vi "Tester - Index First and Last Elements.vi"() -> ()   [LabVIEW 2026, in "RSysUtils Array.lvlib"]
uses:
  RSysUtils Array.lvlib
  fdb9e6c0-975f-44e2-ba30-bd03142f5d50.vi
  b5e11ca3-2994-41fd-9918-31737f74fe56.vi
  f58beb1a-473f-4e9f-bfc2-1733d708c953.vi
  5ddec0b6-ee56-4581-aaaf-1957dd87ccd5.vi
  00215f05-ef31-4d06-8534-21c6b446a682.vi
  7647355d-b8e7-4a93-9c24-6d2a4ea71276.vi
  75d32098-2e7f-4ed5-a06b-df6319fe105d.vi
  2febbabd-baec-49ef-bef3-c8b34b704352.vi
  cc8c92ee-e4ab-4953-afd2-d877638164e4.vi
  083ab0fe-1952-43f6-ad3a-e45cd4cdc5d8.vi
  f95bf693-d319-4365-ae64-cd3e9d60c1cd.vi
  3f8831fb-0eac-4eea-b774-04f899992b81.vi
panel:
  out "Array Out 4":i32[](array[numeric])
  out "Deleted Element 4":i32
  out "Array Out 5":i32[](array[numeric])
  out "Deleted Element 5":i32
  out "Array Out 6":i32[](array[numeric])
  out "Deleted Element 6":i32
  out "Array Out 3":i32[](array[numeric])
  out "Deleted Element 3":i32
  out "Array Out 2":i32[](array[numeric])
  out "Deleted Element 2":i32
  out "Deleted Element 1":i32
  out "Array Out 1":i32[](array[numeric])
  out "Last Element 1":i32
  out "Last Element 2":i32
  out "Last Element 3":i32
  out "First Element 3":i32
  out "First Element 2":i32
  out "First Element 1":i32
  # "Tester\nGet First Element.vim\nGet Last Element.vim"
  # "Get First Element.vim"
  # "Get Last Element.vim"
  # "Delete First Element.vim"
  # "Delete Last Element.vim"
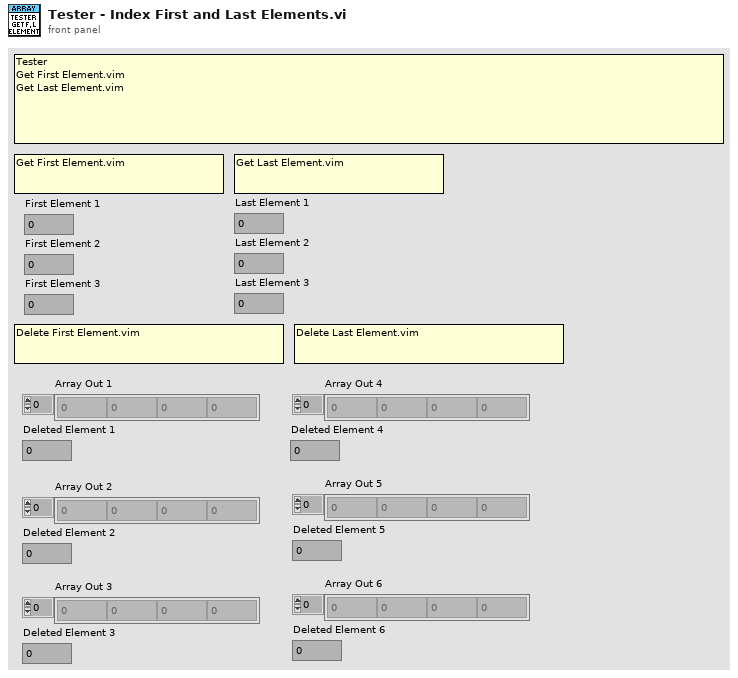
[diagram p1: front panel]
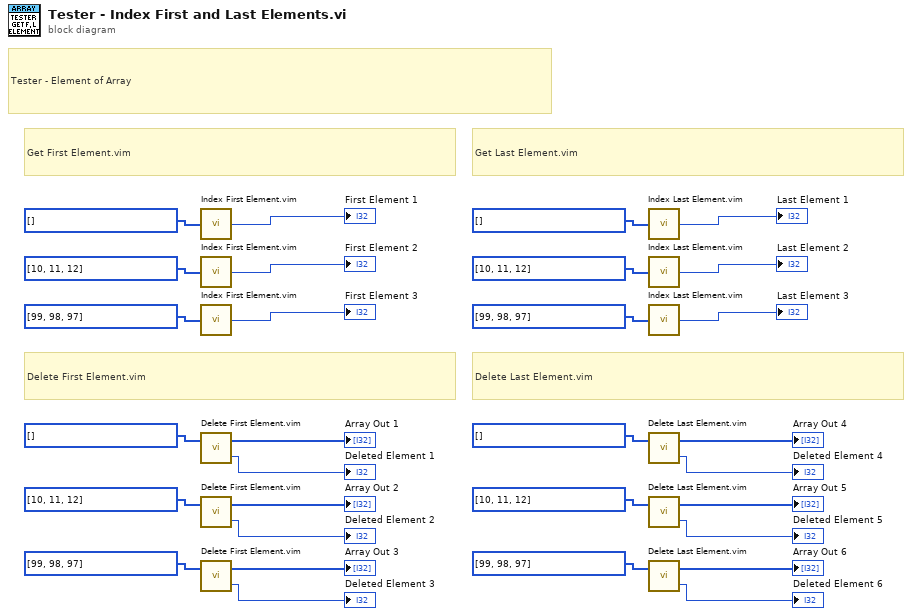
[diagram p0: block diagram]
diagram:
  # "Delete Last Element.vim"
  # "Delete First Element.vim"
  # "Get Last Element.vim"
  # "Get First Element.vim"
  # "Tester - Element of Array"
  n1 = call "Index First Element.vim"("Array"=i32[] []) -> ("First Element"=→"First Element 1":i32)
  n2 = call "Index First Element.vim"("Array"=i32[] [10, 11, 12]) -> ("First Element"=→"First Element 2":i32)
  n3 = call "Index First Element.vim"("Array"=i32[] [99, 98, 97]) -> ("First Element"=→"First Element 3":i32)
  n4 = call "Delete First Element.vim"("Array In"=i32[] []) -> ("Deleted Element"=→"Deleted Element 1":i32, "Array Out"=→"Array Out 1":i32[])  [unwired: 1 in]
  n5 = call "Delete First Element.vim"("Array In"=i32[] [10, 11, 12]) -> ("Deleted Element"=→"Deleted Element 2":i32, "Array Out"=→"Array Out 2":i32[])  [unwired: 1 in]
  n6 = call "Delete First Element.vim"("Array In"=i32[] [99, 98, 97]) -> ("Deleted Element"=→"Deleted Element 3":i32, "Array Out"=→"Array Out 3":i32[])  [unwired: 1 in]
  n7 = call "Index Last Element.vim"("Array"=i32[] []) -> ("Last Element"=→"Last Element 1":i32)
  n8 = call "Index Last Element.vim"("Array"=i32[] [10, 11, 12]) -> ("Last Element"=→"Last Element 2":i32)
  n9 = call "Index Last Element.vim"("Array"=i32[] [99, 98, 97]) -> ("Last Element"=→"Last Element 3":i32)
  n10 = call "Delete Last Element.vim"("Array In"=i32[] []) -> ("Deleted Element"=→"Deleted Element 4":i32, "Array Out"=→"Array Out 4":i32[])  [unwired: 1 in]
  n11 = call "Delete Last Element.vim"("Array In"=i32[] [10, 11, 12]) -> ("Deleted Element"=→"Deleted Element 5":i32, "Array Out"=→"Array Out 5":i32[])  [unwired: 1 in]
  n12 = call "Delete Last Element.vim"("Array In"=i32[] [99, 98, 97]) -> ("Deleted Element"=→"Deleted Element 6":i32, "Array Out"=→"Array Out 6":i32[])  [unwired: 1 in]
